vi "RP1210 Client Connect.vi"(5 "nIsAppPacketizingIncomingMsgs":i16, 6 "lRcvBufferSize":i32, 7 "lTxBufferSize":i32, 8 "error in (no error)":errorcluster, 9 "fpchProtocol":string="CAN:Baud=500", 10 "nDeviceID":i16=1, 11 "hwndClient":u32) -> (0 "error out":errorcluster, 3 "function return":i16)   [LabVIEW 2020, in "cansub_rp1210.lvlib"]
doc: "short __stdcall RP1210_ClientConnect(void *hwndClient, short nDeviceID, char *fpchProtocol,\n long lTxBufferSize, long lRcvBufferSize, short nIsAppPacketizingIncomingMsgs);"
uses:
  cansub_rp1210.lvlib
  cansub_lv64.dll
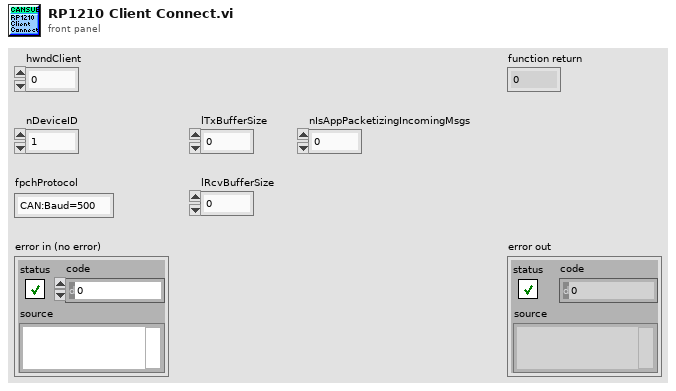
[diagram p1: front panel]
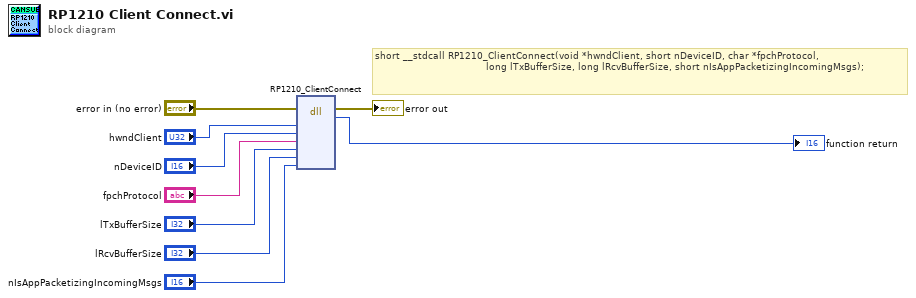
[diagram p0: block diagram]
diagram:
  # "short __stdcall RP1210_ClientConnect(void *hwndClient, short nDeviceID, char *fpchProtocol,\n                                     long lTxBufferSize, long lRcvBufferSize, short nIsAppPacketizingIncomingMsgs);"
  n1 = dll-call lib="C:/cansub-lv/library/cansub_lv*.*" fn="RP1210_ClientConnect"(error in="error in (no error)", "hwndClient"="hwndClient", "nDeviceID"="nDeviceID", "fpchProtocol"="fpchProtocol", "lTxBufferSize"="lTxBufferSize", "lRcvBufferSize"="lRcvBufferSize", "nIsAppPacketizingIncomingMsgs"="nIsAppPacketizingIncomingMsgs") -> (error out=→"error out":errorcluster, "return type"=→"function return":i16)  [unwired: 8 in, 1 out]
